vi "Import Scalars - all.vi"(8 "error in":errorcluster, 11 "FPGA addon refnum in":T3=18446744073709551615 format="%.0x") -> (0 "error out":errorcluster, 2 "imported bitfile scalars out":T1[](array[typedef]), 3 "FPGA addon refnum out":T3=18446744073709551615 format="%.0x")   [LabVIEW 2020, in "Scripting API.lvlib"]
doc: "Imports all of the control and indicator registers contained within. The function operates only on scalar objects. For each control or indicator, a channel will be created within the target FPGA addon, under their respective section (Scalar Inputs or Scalar Outputs). The channel names will correspond to the control and indicator labels within the bitfile.\n\nOnce the import is complete, this function returns an array containing bitfile (control and indicator) registers data, and whether they were imported or not."
uses:
  Scripting API.lvlib
  <vilib>/NI VeriStand/Custom Device API/Custom Device Item Ref.ctl
  TypeDefs/Output Scalar Data.ctl
  Addon/Addon Shared/Types/FPGA Addon Data Type.ctl
  Addon/Addon System Explorer/Types/Channel Type.ctl
  Addon/Addon Shared/Types/FG Action.ctl
  Addon/Addon Shared/SubVIs/Constants.vi
  <vilib>/NI/NI VeriStand Advanced SysDef API/_SubVIs/SysDef.Search.GUID.vi
  <vilib>/NI/NI VeriStand Advanced SysDef API/SysDef API/SysDef.Property.Get.vi
  <vilib>/NI/NI VeriStand Advanced SysDef API/_SubVIs/SysDef.Property.Get.Variant.vi
  <vilib>/NI/NI VeriStand Advanced SysDef API/SysDef API/SysDef.Property.Set.vi
  <vilib>/NI/NI VeriStand Advanced SysDef API/_SubVIs/SysDef.Property.Set.Variant.vi
  Addon/Addon Shared/FPGA Addon Shared.lvlib
  <vilib>/NI/NI VeriStand Advanced SysDef API/SysDef API/Advanced System Definition.lvlib
  Addon/Addon System Explorer/FPGA Addon System Explorer.lvlib
  <vilib>/NI VeriStand/Custom Device API/Custom Device API.lvlib
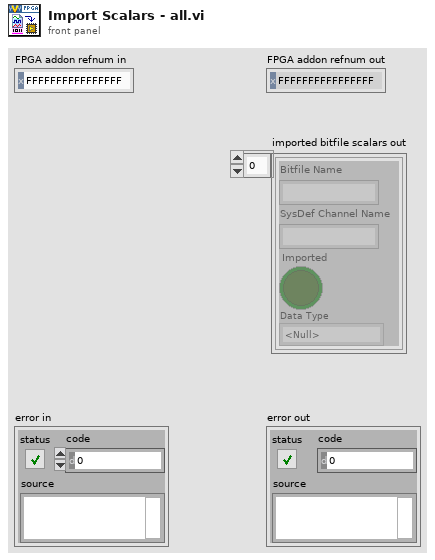
[diagram p1: front panel]
types:
  T1 = typedef "Scripting API.lvlib/Output Scalar Data.ctl" = cluster{"Bitfile Name":string, "SysDef Channel Name":string, "Imported":bool, "Data Type":T2}
  T2 = typedef "FPGA Addon Shared.lvlib/FPGA Addon Data Type.ctl" = enum8{"<Null>", "I8", "I16", "I32", "I64", "U8", "U16", "U32", "U64", "SGL", "Boolean", "Analog PWM In Settings", "Analog PWM In", "Digital PWM In Settings", "Digital PWM In", "Digital PWM Out", "Sine Out", "FXP", "FXP+/-24.5", "FXP+/-16.5", "FXP+/-32.8", "FXP+/-64.32", "FXP+/-16.7", "FXP+/-20.5", "FXP+/-27.5", "FXP+/-32.16", "FXP+16.3", "FXP+18.3", "Digital Static In", "Digital Static Out", "Digital Static In Settings", "Digital WSS Out", "Quad Encoder Settings", "Quad Encoder In", "Group"}
  T3 = typedef "Custom Device API.lvlib/Custom Device Item Ref.ctl" = u64
  T4 = typedef "FPGA Addon System Explorer.lvlib/Channel Type.ctl" = enum16{"Write Channel", "Read Channel", "Write Waveform", "Read Waveform"}
  T5 = typedef "FPGA Addon Shared.lvlib/FG Action.ctl" = enum8{"GET", "SET"}
  T6 = typedef "FPGA Addon Shared.lvlib/Register Information.ctl" = cluster{"Name":string, "Data Type":T2, "Default Value":variant, "Attributes":variant}
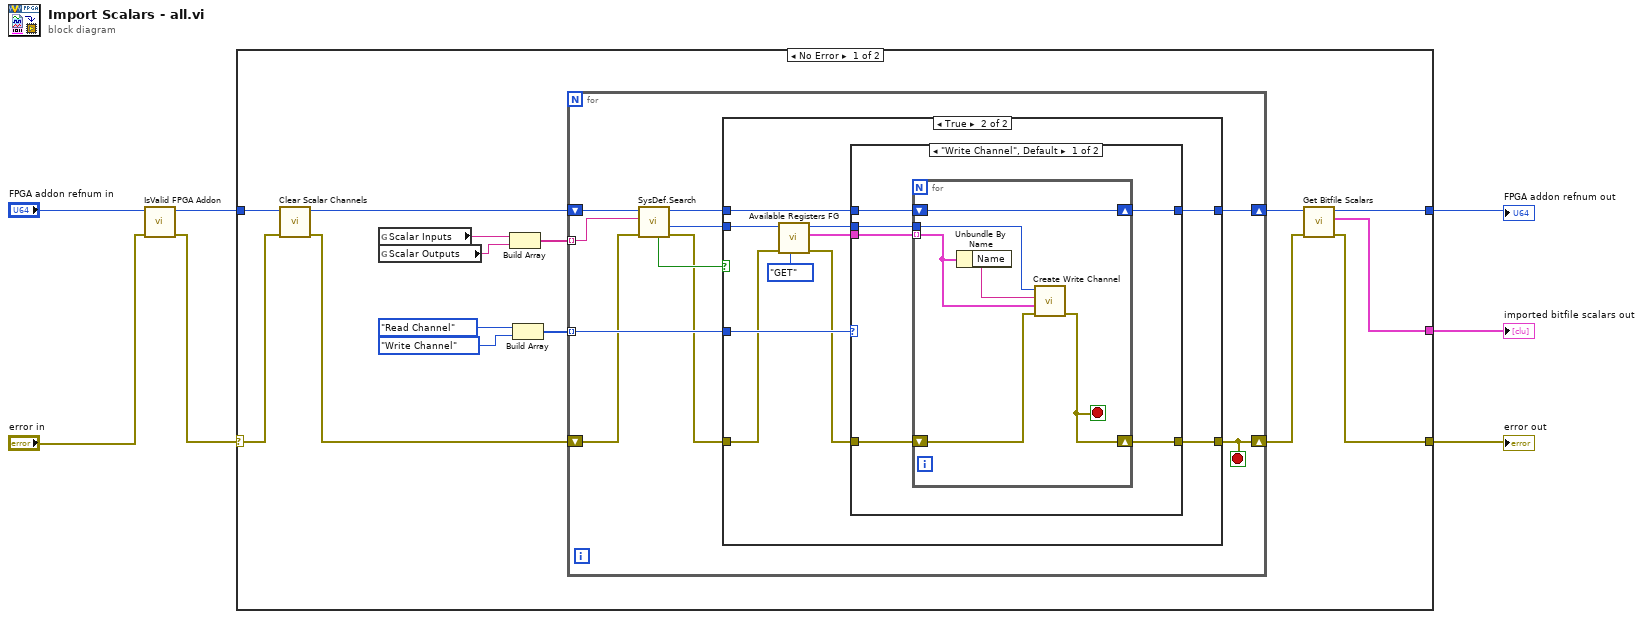
[diagram p0: block diagram]
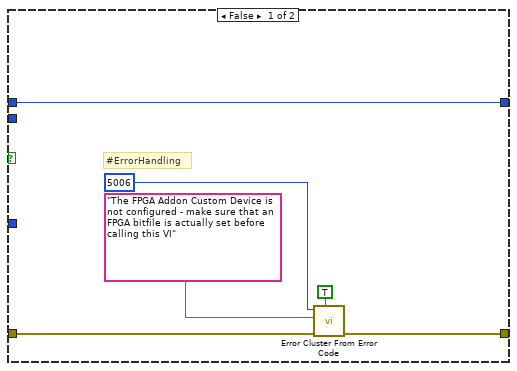
[diagram p2: hidden frame]
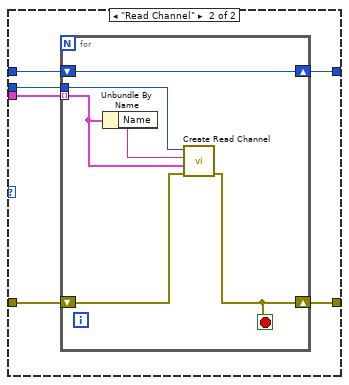
[diagram p3: hidden frame]
diagram:
  n1 = call "IsValid FPGA Addon.vi"("error in"="error in", "FPGA Addon refnum in"="FPGA addon refnum in") -> ("error out"=w5:errorcluster, "FPGA Addon refnum out"=w4:T3)  [unwired: 8 in]
  n2 = case shown="No Error" w5 {
    selector: w5 -> [w9 w74]
    tunnel: w4 -> [w11 w73]
    tunnel: [w15 w73] -> w3
    tunnel: [w13 w74] -> w2
    tunnel: [w12 _] -> w1
    frame No Error {
      n3 = call "Clear Scalar Channels.vi"("error in"=w9, "FPGA Addon refnum in"=w11) -> ("error out"=w8:errorcluster, "FPGA Addon refnum out"=w10:T3)  [unwired: 8 in]
      n4 = global read "Constants.vi" "Scalar Inputs"() -> (w22:string)
      n5 = global read "Constants.vi" "Scalar Outputs"() -> (w21:string)
      n6 = Build Array(w22, w21) -> (w20:string[])
      n7 = Build Array(Channel_Type."Read Channel" ("Action"), Channel_Type."Write Channel" ("Action")) -> (w17:T4[])
      n8 = for {
        tunnel: w20 -> [w31] mode=indexing
        shift-right: [w24] -> w16
        shift-left: w10 -> [w32]
        tunnel: w17 -> [w28] mode=indexing
        shift-right: [w23] -> w14
        shift-left: w8 -> [w27]
        stop <- w23 stop-if-true
        n9 = call-poly <vilib>:"SysDef.Search.vi"("error in (no error)"=w27, "GUID"=w31, "nodeID"=w32) -> ("error out"=w26:errorcluster, "Value out"=w29:u64, "nodeID out"=w25:u64, "Found?"=w30:bool)  [unwired: 5 in]
        n10 = case shown="True" w30 {
          tunnel: w29 -> [_ w47]
          tunnel: w28 -> [_ w44]
          tunnel: w26 -> [w35 w43]
          tunnel: [w34 w41] -> w23
          tunnel: w25 -> [w38 w40]
          tunnel: [w38 w39] -> w24
          frame False {
            # "#ErrorHandling"
            n11 = call <vilib>:"Error Cluster From Error Code.vi"("show call chain? (False)"=TRUE, "error in (no error)"=w35, "error message (\"\")"="The FPGA Addon Custom Device is not configured - make sure that an FPGA bitfile is actually set before calling this VI" ("error message (\"\")"), "error code (0)"=5006) -> ("error out"=w34:errorcluster)  [unwired: 5 in]
          }
          frame True {
            n12 = call "Available Registers FG.vi"("Action"=FG_Action."GET", "error in (no error)"=w43, "Item Ref"=w47) -> ("error out"=w42:errorcluster, "Available Registers"=w46:T6[], "Item Ref out"=w45:T3)  [unwired: 6 in]
            n13 = case shown="\"Write Channel\", Default" w44 {
              tunnel: w46 -> [w51 w66]
              tunnel: w45 -> [w52 w65]
              tunnel: w42 -> [w54 w64]
              tunnel: [w53 w63] -> w41
              tunnel: w40 -> [w50 w62]
              tunnel: [w49 w61] -> w39
              frame "Write Channel", Default {
                n14 = for {
                  tunnel: w51 -> [w58] mode=indexing
                  tunnel: w52 -> [w60]
                  shift-right: [w55] -> w53
                  shift-left: w54 -> [w57]
                  shift-right: [w56] -> w49
                  shift-left: w50 -> [w56]
                  stop <- w55 stop-if-true
                  n15 = Unbundle By Name(w58) -> ("Name"=w59:string)
                  n16 = call "Create Write Channel.vi"("error in (no error)"=w57, "Cluster"=w58, "Bitfile Name"=w59, "Item Ref in"=w60) -> ("error out"=w55:errorcluster)  [unwired: 7 in]
                }
              }
              frame "Read Channel" {
                n17 = for {
                  tunnel: w66 -> [w70] mode=indexing
                  tunnel: w65 -> [w71]
                  shift-right: [w67] -> w63
                  shift-left: w64 -> [w69]
                  shift-right: [w68] -> w61
                  shift-left: w62 -> [w68]
                  stop <- w67 stop-if-true
                  n18 = Unbundle By Name(w70) -> ("Name"=w72:string)
                  n19 = call "Create Read Channel.vi"("error in (no error)"=w69, "Channel"=w70, "Bitfile Name"=w72, "Item Ref in"=w71) -> ("error out"=w67:errorcluster)  [unwired: 7 in]
                }
              }
            }
          }
        }
      }
      n20 = call "Get Bitfile Scalars.vi"("error in"=w14, "FPGA addon refnum in"=w16) -> ("error out"=w13:errorcluster, "bitfile scalars out"=w12:T1[], "FPGA addon refnum out"=w15:T3)  [unwired: 7 in]
    }
    frame Error {
    }
  }
  "error out" <- w2
  "FPGA addon refnum out" <- w3
  "imported bitfile scalars out" <- w1
